vi "RemoteVI Control Children.vi"(0 "Control":refnum<vi>, 11 "error in":errorcluster) -> (4 "Children":refnum<vi>[](array[refnum]), 15 "error out":errorcluster)   [LabVIEW 2020, in "RemoteVI.lvlib"]
doc: "The controls one level inside Control that a user can see now: the controls on the SELECTED page of a tab control (its value, read as the first Val of its XML), the elements of a cluster, nothing for any other control. For RemoteVI Read Tips.vi. A control that is neither a tab control nor a cluster is the normal case, so the failed casts are not errors; errors of the property reads go to error out."
uses:
  RemoteVI.lvlib
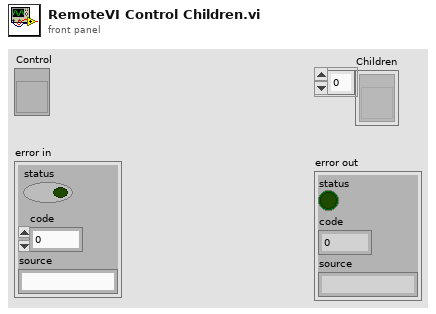
[diagram p1: front panel]
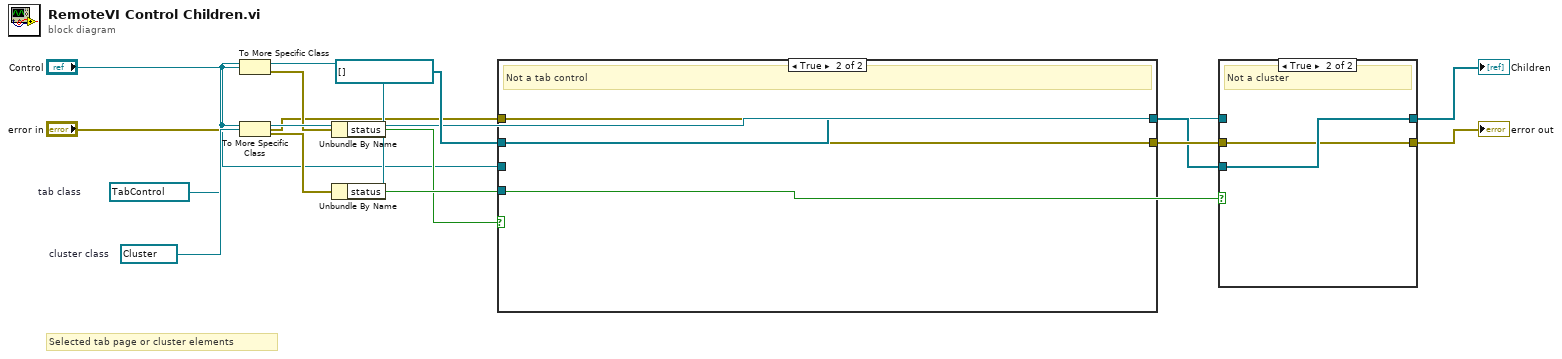
[diagram p0: block diagram]
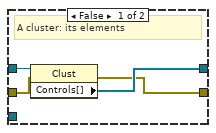
[diagram p2: hidden frame]
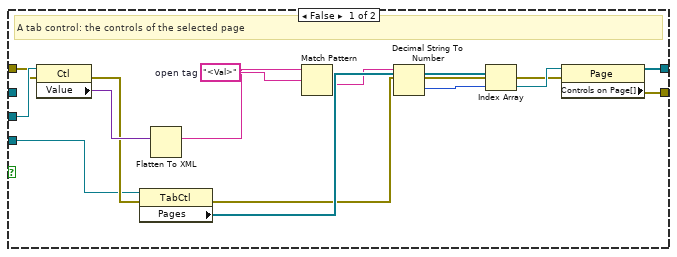
[diagram p3: hidden frame]
diagram:
  w4 = refnum<vi> refnum  # cluster class
  w3 = refnum<vi> refnum  # tab class
  # "Selected tab page or cluster elements"
  n1 = To More Specific Class(target class=w3, reference="Control") -> (specific class reference=w5:refnum<vi>, error out=w6:errorcluster)  [unwired: 1 in]
  n2 = To More Specific Class(target class=w4, reference="Control") -> (specific class reference=w7:refnum<vi>, error out=w8:errorcluster)  [unwired: 1 in]
  n3 = Unbundle By Name(w6) -> ("status"=w9:bool)
  n4 = Unbundle By Name(w8) -> ("status"=w10:bool)
  n5 = case shown="True" w9 {
    tunnel: "error in" -> [w17 w30]
    tunnel: refnum<vi>[] [] -> [_ w31]
    tunnel: "Control" -> [w18 _]
    tunnel: w5 -> [w16 _]
    tunnel: [w29 w31] -> w12
    tunnel: [w28 w30] -> w13
    frame False {
      w22 = "<Val>"  # open tag
      # "A tab control: the controls of the selected page"
      n6 = property class="Ctl"(reference=w18, error in=w17) -> (error out=w19:errorcluster, "Value"=w20:variant)  [unwired: 1 out]
      n7 = property class="TabCtl"(reference=w16, error in=w19) -> (error out=w25:errorcluster, "Pages"=w26:refnum<vi>[])  [unwired: 1 out]
      n8 = Flatten To XML(6:w20) -> (2:w21:string)
      n9 = Match Pattern(string=w21, regular expression=w22) -> (after substring=w23:string)  [unwired: 1 in, 3 out]
      n10 = Decimal String To Number(string=w23) -> (number=w24:i32)  [unwired: 2 in, 1 out]
      n11 = Index Array(array=w26, index=w24) -> (element=w27:refnum<vi>)
      n12 = property class="Page"(reference=w27, error in=w25) -> (error out=w28:errorcluster, "Controls on Page[]"=w29:refnum<vi>[])  [unwired: 1 out]
    }
    frame True {
      # "Not a tab control"
    }
  }
  n13 = case shown="True" w10 {
    tunnel: w7 -> [w32 _]
    tunnel: w13 -> [w33 w36]
    tunnel: w12 -> [_ w37]
    tunnel: [w35 w37] -> w14
    tunnel: [w34 w36] -> w15
    frame False {
      # "A cluster: its elements"
      n14 = property class="Clust"(reference=w32, error in=w33) -> (error out=w34:errorcluster, "Controls[]"=w35:refnum<vi>[])  [unwired: 1 out]
    }
    frame True {
      # "Not a cluster"
    }
  }
  "Children" <- w14
  "error out" <- w15
